vi "probeN.vi"(0 "x":dbl=1.0) -> (4 "out":cluster{"A":dbl, "Stop":bool}, 15 "error out":errorcluster)   [LabVIEW 2026]
doc: "p"
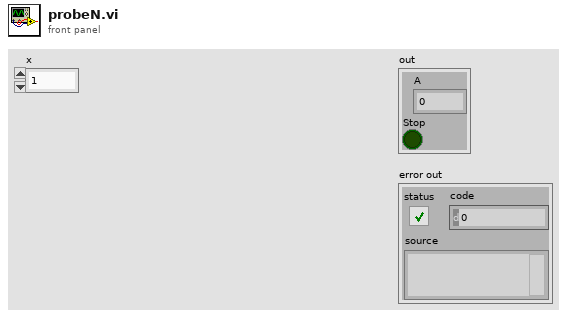
[diagram p1: front panel]
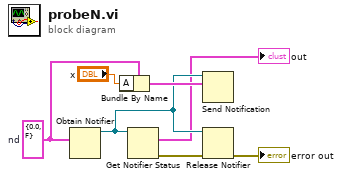
[diagram p0: block diagram]
diagram:
  w6 = cluster{"A":dbl, "Stop":bool} {"A"=0.0, "Stop"=FALSE}  # nd
  n1 = Obtain Notifier(notification data type=w6) -> (notifier out=w4:refnum<notifier>)  [unwired: 3 in, 2 out]
  n2 = Bundle By Name(cluster=w6, "A"="x") -> (w5:cluster{"A":dbl, "Stop":bool})
  n3 = Get Notifier Status(notifier=w4) -> (current notification=→"out":cluster{"A":dbl, "Stop":bool}, error out=w3:errorcluster)  [unwired: 1 in, 3 out]
  n4 = Send Notification(notification=w5, notifier=w4) -> ()  [unwired: 1 in, 2 out]
  n5 = Release Notifier(notifier=w4, error in (no error)=w3) -> (error out=→"error out":errorcluster)  [unwired: 1 in, 2 out]
